vi "Initialize Display Size.vi"(8 "error in (no error)":errorcluster, 9 "Height":u32=20, 10 "Width":u32=120, 11 "Display ref":refnum<vi>) -> (0 "error out":errorcluster, 3 "Display":picture)   [LabVIEW 2018, in "Pass Fail Display.lvlib"]
uses:
  Pass Fail Display.lvlib
  <vilib>/Utility/miscctls.llb/LVBoundsTypeDef.ctl
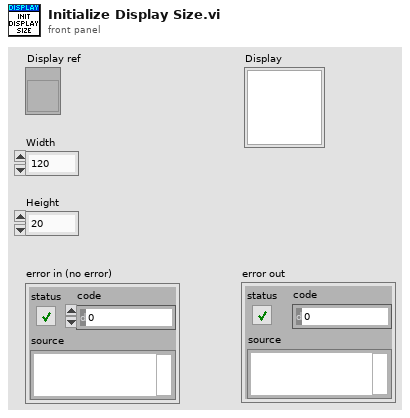
[diagram p1: front panel]
types:
  T1 = typedef "LVBoundsTypeDef.ctl" = cluster{"Width":u32, "Height":u32}
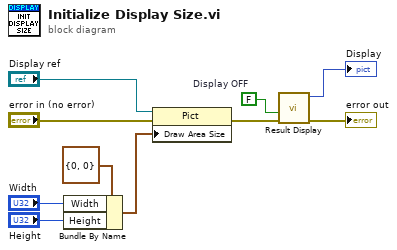
[diagram p0: block diagram]
diagram:
  w5 = FALSE  # Display OFF
  n1 = Bundle By Name(cluster=T1 {"Width"=0, "Height"=0} ("Draw Area Size"), "Width"="Width", "Height"="Height") -> (w10:T1)
  n2 = property class="Pict"(reference="Display ref", error in="error in (no error)", "Draw Area Size"=w10) -> (error out=w4:errorcluster)  [unwired: 1 out]
  n3 = call "Result Display.vi"("error in (no error)"=w4, "Display ON/OFF"=w5) -> ("error out"=→"error out":errorcluster, "Result Display"=→"Display":picture)  [unwired: 8 in]
